vi "To XML.vi"(8 "error in (no error)":errorcluster, 9 "Parent":refnum<k20>, 10 "Document":refnum<k20>, 11 "Class in":refnum<class "Class.lvclass">) -> (0 "error out":errorcluster)   [LabVIEW 2017, in "Cobertura.lvlib" / "Class.lvclass"]
uses:
  Class.lvclass
  Class.lvclass/Class.ctl
  <vilib>/xml/Close Reference(Node).vi
  Method/Method.lvclass
  <resource>/objmgr/DOMUserDefRef.rc
  <vilib>/xml/NI_XML.lvlib
  Cobertura.lvlib
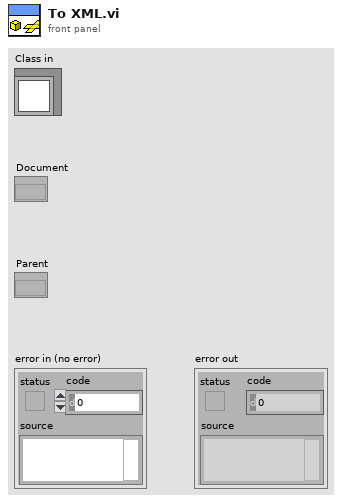
[diagram p1: front panel]
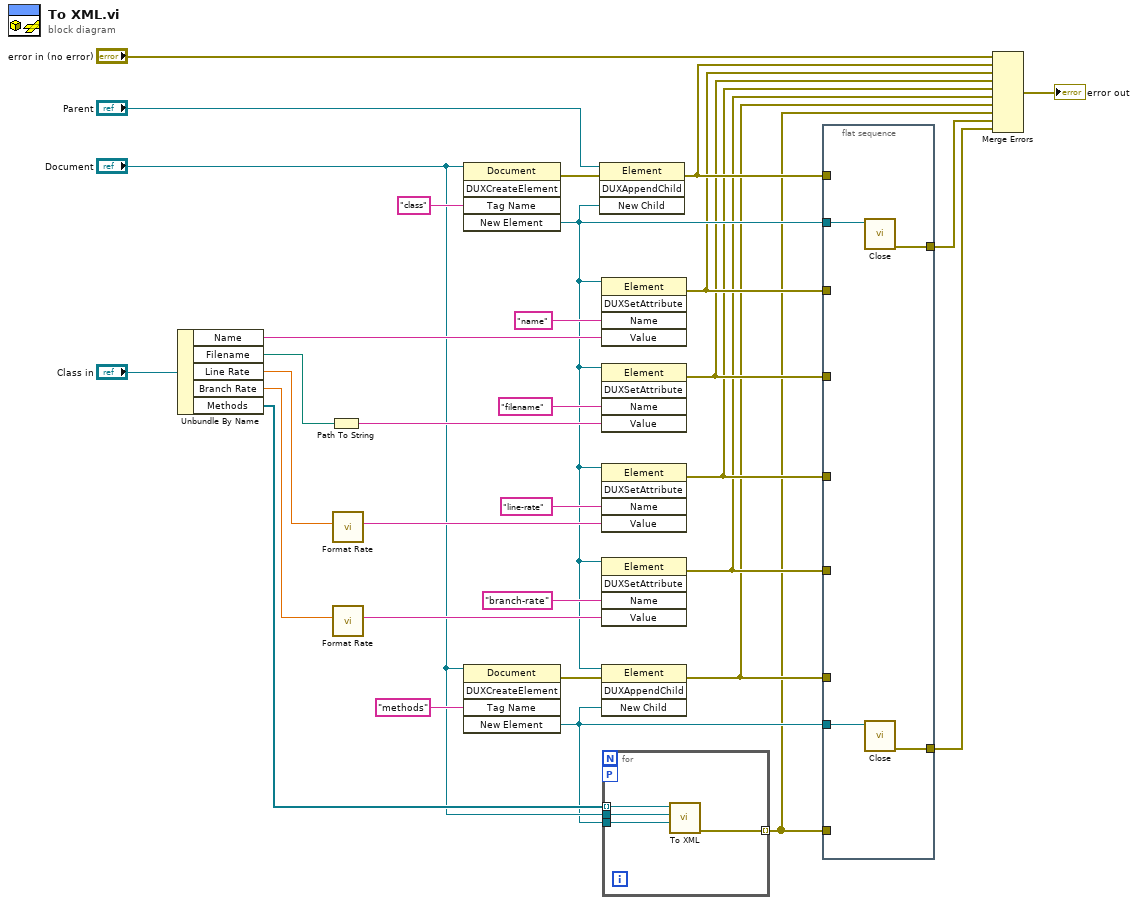
[diagram p0: block diagram]
diagram:
  n1 = Unbundle By Name("Class in") -> ("Name"=w24:string, "Filename"=w22:path, "Line Rate"=w2:dbl, "Branch Rate"=w1:dbl, "Methods"=w19:refnum<class "Method.lvclass">[])
  n2 = Path To String(path=w22) -> (string=w21:string)
  n3 = call "Format Rate.vi"("Rate"=w2) -> ("String"=w30:string)  [unwired: 10 in]
  n4 = call "Format Rate.vi"("Rate"=w1) -> ("String"=w28:string)  [unwired: 10 in]
  n5 = invoke class="Document" method="DUXCreateElement"(reference="Document", "Tag Name"="class") -> (error out=w16:errorcluster, "New Element"=w15:refnum<k20>)  [unwired: 3 in, 3 out]
  n6 = invoke class="Document" method="DUXCreateElement"(reference="Document", "Tag Name"="methods") -> (error out=w17:errorcluster, "New Element"=w14:refnum<k20>)  [unwired: 3 in, 3 out]
  n7 = invoke class="Element" method="DUXAppendChild"(reference="Parent", error in=w16, "New Child"=w15) -> (error out=w13:errorcluster)  [unwired: 1 in, 3 out]
  n8 = invoke class="Element" method="DUXSetAttribute"(reference=w15, "Name"="name", "Value"=w24) -> (error out=w12:errorcluster)  [unwired: 2 in, 4 out]
  n9 = invoke class="Element" method="DUXSetAttribute"(reference=w15, "Name"="filename", "Value"=w21) -> (error out=w11:errorcluster)  [unwired: 2 in, 4 out]
  n10 = invoke class="Element" method="DUXSetAttribute"(reference=w15, "Name"="line-rate", "Value"=w30) -> (error out=w10:errorcluster)  [unwired: 2 in, 4 out]
  n11 = invoke class="Element" method="DUXSetAttribute"(reference=w15, "Name"="branch-rate", "Value"=w28) -> (error out=w9:errorcluster)  [unwired: 2 in, 4 out]
  n12 = invoke class="Element" method="DUXAppendChild"(reference=w15, error in=w17, "New Child"=w14) -> (error out=w8:errorcluster)  [unwired: 1 in, 3 out]
  n13 = for {
    tunnel: w19 -> [w36] mode=indexing
    tunnel: "Document" -> [w35]
    tunnel: w14 -> [w34]
    workers-P: _ -> [_]
    tunnel: [w33] -> w7 mode=indexing
    n14 = call-dynamic "To XML.vi"("Parent"=w34, "Document"=w35, "Method in"=w36) -> ("error out"=w33:errorcluster)  [unwired: 8 in]
  }
  n15 = flat-sequence {
    tunnel: w15 -> [w40]
    tunnel: w14 -> [w39]
    tunnel: w7 -> [_]
    tunnel: w8 -> [_]
    tunnel: w9 -> [_]
    tunnel: w10 -> [_]
    tunnel: w11 -> [_]
    tunnel: w12 -> [_]
    tunnel: w13 -> [_]
    tunnel: [w38] -> w4
    tunnel: [w37] -> w3
    frame #0 {
      n16 = call-poly <vilib>:"Close.vi"("node"=w40) -> ("error out"=w38:errorcluster)  [unwired: 8 in]
      n17 = call-poly <vilib>:"Close.vi"("node"=w39) -> ("error out"=w37:errorcluster)  [unwired: 8 in]
    }
  }
  n18 = Merge Errors("error in (no error)", w13, w12, w11, w10, w9, w8, w7, w4, w3) -> (→"error out":errorcluster)
